vi "SetValueByHierarchicalPath.vi"(0 "VI Reference In":refnum<vi>, 2 "delimiter (>>)":string=">>", 5 "Control Path":string, 7 "Hierarchical Path":string, 11 "Error In":errorcluster) -> (4 "VI Reference Out":refnum<vi>, 15 "Error Out":errorcluster)   [LabVIEW 2016, in "Drona.lvlib" / "ControlValue.lvlib" / "StimulusTree.lvlib"]
doc: "Sets value(signaling) for the tree control whose item name is specified as a hierarchical path.\n\nHierarchical path represent their corresponding parents of an item from its origin. Use the delimiters '>>' between each hierarchy in the path.\n\nFor example to select the item 'Child3', give the hierarchical path as \"<b>Parent1</b>(top level parent in tree)<b>>>Child1</b>(children for parent1)<b>>>Child2</b>(children for child1)<b>>>Child3</b>(children for child2)\"\n\nThe input control name is given as a string , incase of path, use delimiters inbetween the path."
uses:
  StimulusTree.lvlib
  <vilib>/Utility/error.llb/Error Cluster From Error Code.vi
  <vilib>/ErrorRing/Error Ring.xnode
  Drona.lvlib
  Get/GetControlRef/GetControlRef.lvlib
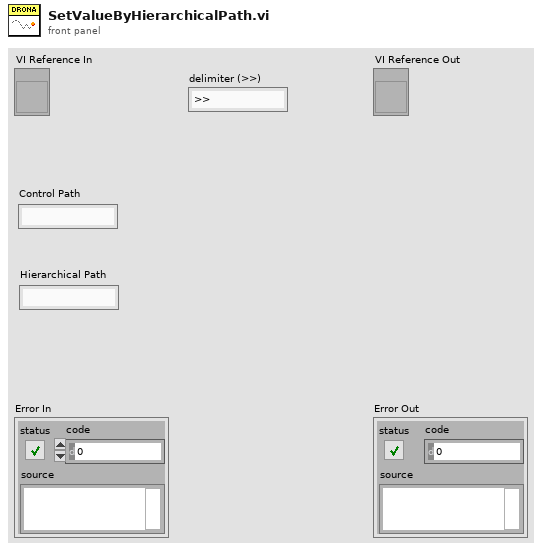
[diagram p1: front panel]
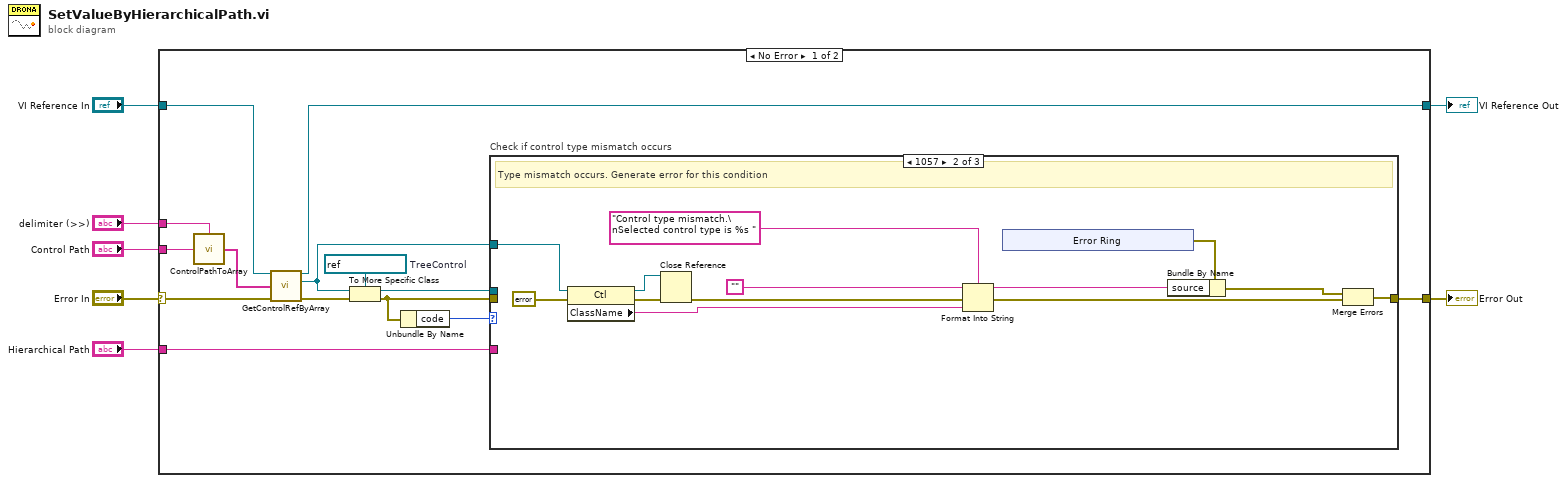
[diagram p0: block diagram]
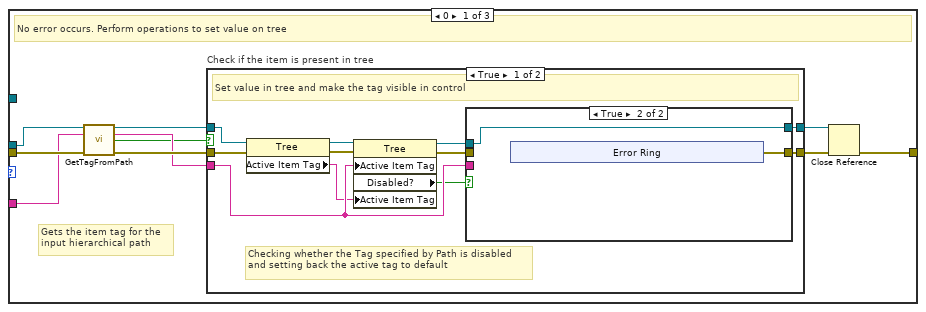
[diagram p2: hidden frame]
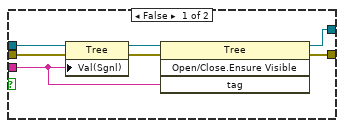
[diagram p3: hidden frame]
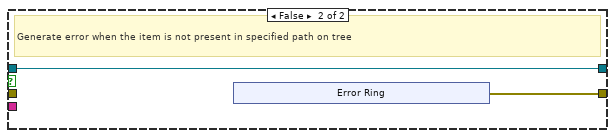
[diagram p4: hidden frame]
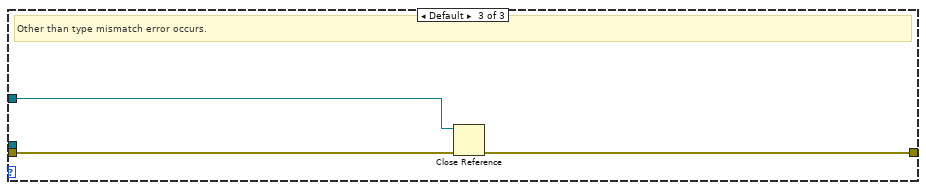
[diagram p5: hidden frame]
diagram:
  n1 = case shown="No Error" "Error In" {
    selector: "Error In" -> [w18 w86]
    tunnel: [w8 w86] -> w6
    tunnel: "VI Reference In" -> [w17 w85]
    tunnel: "Control Path" -> [w20 _]
    tunnel: [w14 w85] -> w3
    tunnel: "delimiter (>>)" -> [w19 _]
    tunnel: "Hierarchical Path" -> [w9 _]
    frame No Error {
      w21 = refnum<vi> refnum  # TreeControl
      n2 = call "ControlPathToArray.vi"("Control Name"=w20, "delimiter (>>)"=w19) -> ("Control Path"=w16:string[])
      n3 = call "GetControlRefByArray.vi"("VI Reference In"=w17, "Control Path"=w16, "error In"=w18) -> ("VI Reference Out"=w14:refnum<vi>, "Ctl Refnum"=w13:refnum<vi>, "error out"=w15:errorcluster)  [unwired: 10 in]
      n4 = To More Specific Class(target class=w21, reference=w13, error in=w15) -> (specific class reference=w12:refnum<vi>, error out=w11:errorcluster)
      n5 = Unbundle By Name(w11) -> ("code"=w10:i32)
      n6 = case "Check if control type mismatch occurs" shown="1057" w10 {
        tunnel: [w31 w66 w83] -> w8
        tunnel: w12 -> [w26 _ _]
        tunnel: w13 -> [_ w76 w82]
        tunnel: w11 -> [w28 _ w84]
        tunnel: w9 -> [w25 _ _]
        frame 0 {
          # "Gets the item tag for the \ninput hierarchical path"
          # "No error occurs. Perform operations to set value on tree"
          n7 = call "GetTagFromPath.vi"("Tree Ref In"=w26, "Hierarchical Path"=w25, "Error In"=w28) -> ("Tree Ref Out"=w24:refnum<vi>, "Item Tag"=w23:string, "Item Found?"=w22:bool, "Error Out"=w27:errorcluster)  [unwired: 9 in]
          n8 = case "Check if the item is present in tree" shown="True" w22 {
            tunnel: [w42 w58] -> w30
            tunnel: [w41 w57] -> w29
            tunnel: w24 -> [w35 w57]
            tunnel: w23 -> [w38 _]
            tunnel: w27 -> [w36 _]
            frame True {
              # "Checking whether the Tag specified by Path is disabled and setting back the active tag to default"
              # "Set value in tree and make the tag visible in control"
              n9 = property class="Tree"(reference=w35, error in=w36) -> (reference out=w34:refnum<vi>, error out=w33:errorcluster, "Active Item Tag"=w32:string)
              n10 = property class="Tree"(reference=w34, error in=w33, "Active Item Tag"=w38, "Active Item Tag"=w32) -> (reference out=w40:refnum<vi>, error out=w39:errorcluster, "Disabled?"=w37:bool)
              n11 = case shown="True" w37 {
                tunnel: [w48 w51] -> w42
                tunnel: [w46 w50] -> w41
                tunnel: w40 -> [w45 w50]
                tunnel: w39 -> [w44 _]
                tunnel: w38 -> [w43 _]
                frame False {
                  n12 = property class="Tree"(reference=w45, error in=w44, "Val(Sgnl)"=w43) -> (reference out=w47:refnum<vi>, error out=w49:errorcluster)
                  n13 = invoke class="Tree" method="Open/Close.Ensure Visible"(reference=w47, error in=w49, "tag"=w43) -> (reference out=w46:refnum<vi>, error out=w48:errorcluster)  [unwired: 1 in, 2 out]
                }
                frame True {
                  n14 = xnode "Error Ring"() -> ("error out"=w51:errorcluster)
                }
              }
            }
            frame False {
              # "Generate error when the item is not present in specified path on tree"
              n15 = xnode "Error Ring"() -> ("error out"=w58:errorcluster)
            }
          }
          n16 = Close Reference(reference=w29, error in (no error)=w30) -> (error out=w31:errorcluster)
        }
        frame 1057 {
          # "Type mismatch occurs. Generate error for this condition"
          n17 = property class="Ctl"(reference=w76, error in=errorcluster {"status"=FALSE, "code"=0, "source"=""} ("error out")) -> (reference out=w64:refnum<vi>, error out=w75:errorcluster, "ClassName"=w72:string)
          n18 = Close Reference(reference=w64, error in (no error)=w75) -> (error out=w65:errorcluster)
          n19 = Format Into String(format string="Control type mismatch.\nSelected control type is %s ", initial string="", error in=w65, w72) -> (resulting string=w69:string, error out=w67:errorcluster)
          n20 = xnode "Error Ring"() -> ("error out"=w70:errorcluster)
          n21 = Bundle By Name(cluster=w70, "source"=w69) -> (w68:errorcluster)
          n22 = Merge Errors(w68, w67) -> (w66:errorcluster)
        }
        frame Default {
          # "Other than type mismatch error occurs."
          n23 = Close Reference(reference=w82, error in (no error)=w84) -> (error out=w83:errorcluster)
        }
      }
    }
    frame Error {
    }
  }
  "Error Out" <- w6
  "VI Reference Out" <- w3
